vi "CSM - Running Log - DebugTool.vi"(10 "Current Module(\"\" to generate an ID)":string="Debug-LogViewer") -> ()   [LabVIEW 2017]
doc: "CSM overall program running log real-time viewer."
uses:
  Utility/_support/Periodic String Filter Level.ctl
  Utility/Periodic String Filter Setting.ctl
  _Shared/Change Speed Counter.vi
  _Shared/Rising Edge.vi
  _Shared/Debounced Signal.vi
  Communicable State Machine.lvlib
  _Shared/CSM Shared.lvlib
  _Support/csm-tool-support.lvlib
  _csmHelper/API with lvcsm Support/CSM-Helper API with lvcsm Support.lvlib
  addons/Logger/CSM File Logger.lvlib
  _ui/csm-ui-support.lvlib
panel:
  in  "Record.Stop":bool
  in  "Record.Start":bool
  in  "Clear":bool
  in  "BackTop":bool
  in  "Toolbar.History Length(char)":i32=50000 caption="History(char)" min=1000 max=100000000 step=1
  in  "Peroid Logs":bool
  out "State History":string
  in  "Tab":enum32{"Error History", "Broadcast Registry"}(tab)
  out "Error History":string
  out "Broadcast Registry":string[][](table)
  out "LogInQ":i32 caption="LogInQ:"
  out "log handling Speed(#/s)":dbl caption="log handling Speed(#/s):"
  out "LogInQ change(#/s)":dbl caption="LogInQ change(#/s):"
  out "Level":T1 caption="Level:"
  in  "Stop":bool
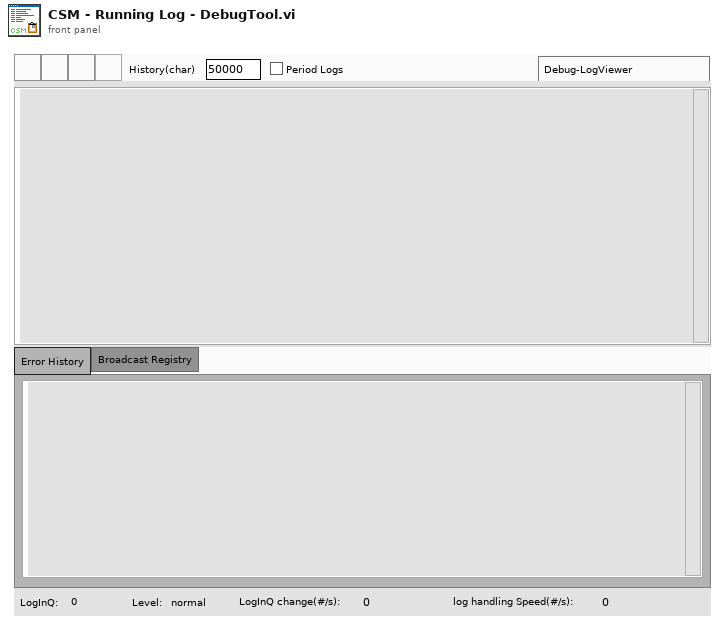
[diagram p1: front panel]
types:
  T1 = typedef "Communicable State Machine.lvlib/Periodic String Filter Level.ctl" = enum16{"normal", "L1", "L2", "L3", "L4"}
  T2 = typedef "Communicable State Machine.lvlib/Periodic String Filter Setting.ctl" = cluster{"threashold(#/s)":dbl, "Check Peroid(s)":dbl}
  T3 = typedef "Communicable State Machine.lvlib/_CSM_GlobalLog_MSG.ctl" = cluster{"Name (\"\" to Use UUID)":string, "Current State":string, "Arguments":string, "Source Message":T4, "Source Module":string, "Complete(T)/Start(F)":bool, "LogType":T5, "Time Stamp":timestamp}
  T4 = typedef "Communicable State Machine.lvlib/_CSM_Response Source Message.ctl" = cluster{"‘State":string, "’Arguments":string, "’Error":errorcluster}
  T5 = typedef "Communicable State Machine.lvlib/_CSM_GlobalLog_MSG_TYPE.ctl" = enum16{"User Log", "State Change", "Status", "Interrupt", "Register", "Unregister", "Error Log", "Module Created", "Module Destroyed", "Async Message", "No-Rep Async Message", "Sync Message"}
  T6 = enum32{"Invalid", "Standard", "Closed", "Hidden", "Minimized", "Maximized"}
  T7 = enum32{"invalid app kind", "Development System", "Run Time System", "Student Edition", "Embedded LabVIEW", "Evaluation", "Custom"}
  T8 = typedef "LVPoint32TypeDef.ctl" = cluster{"Horizontal":i32, "Vertical":i32}
  T9 = cluster{"Shift":bool, "Ctrl":bool, "Alt":bool, "Cmd":bool, "Opt":bool}
  T10 = cluster{"Core":cluster{"Current VI Reference":refnum<vi>, "Close Panel on Exit?":bool}, "Toolbar.Advance":refnum<vi>[], "LoggerWatchDogQueue":refnum<queue>, "LogFile":path}
  T11 = cluster{"Current VI Reference":refnum<vi>, "Close Panel on Exit?":bool}
  T12 = typedef "Communicable State Machine.lvlib/CSM - Broadcast Message Type.ctl" = enum16{"<Null>", "Status", "Interrupt"}
  T13 = cluster{string, "Name":string, "Target CSM":string, "Target State":string, "Register Type":T12}[]
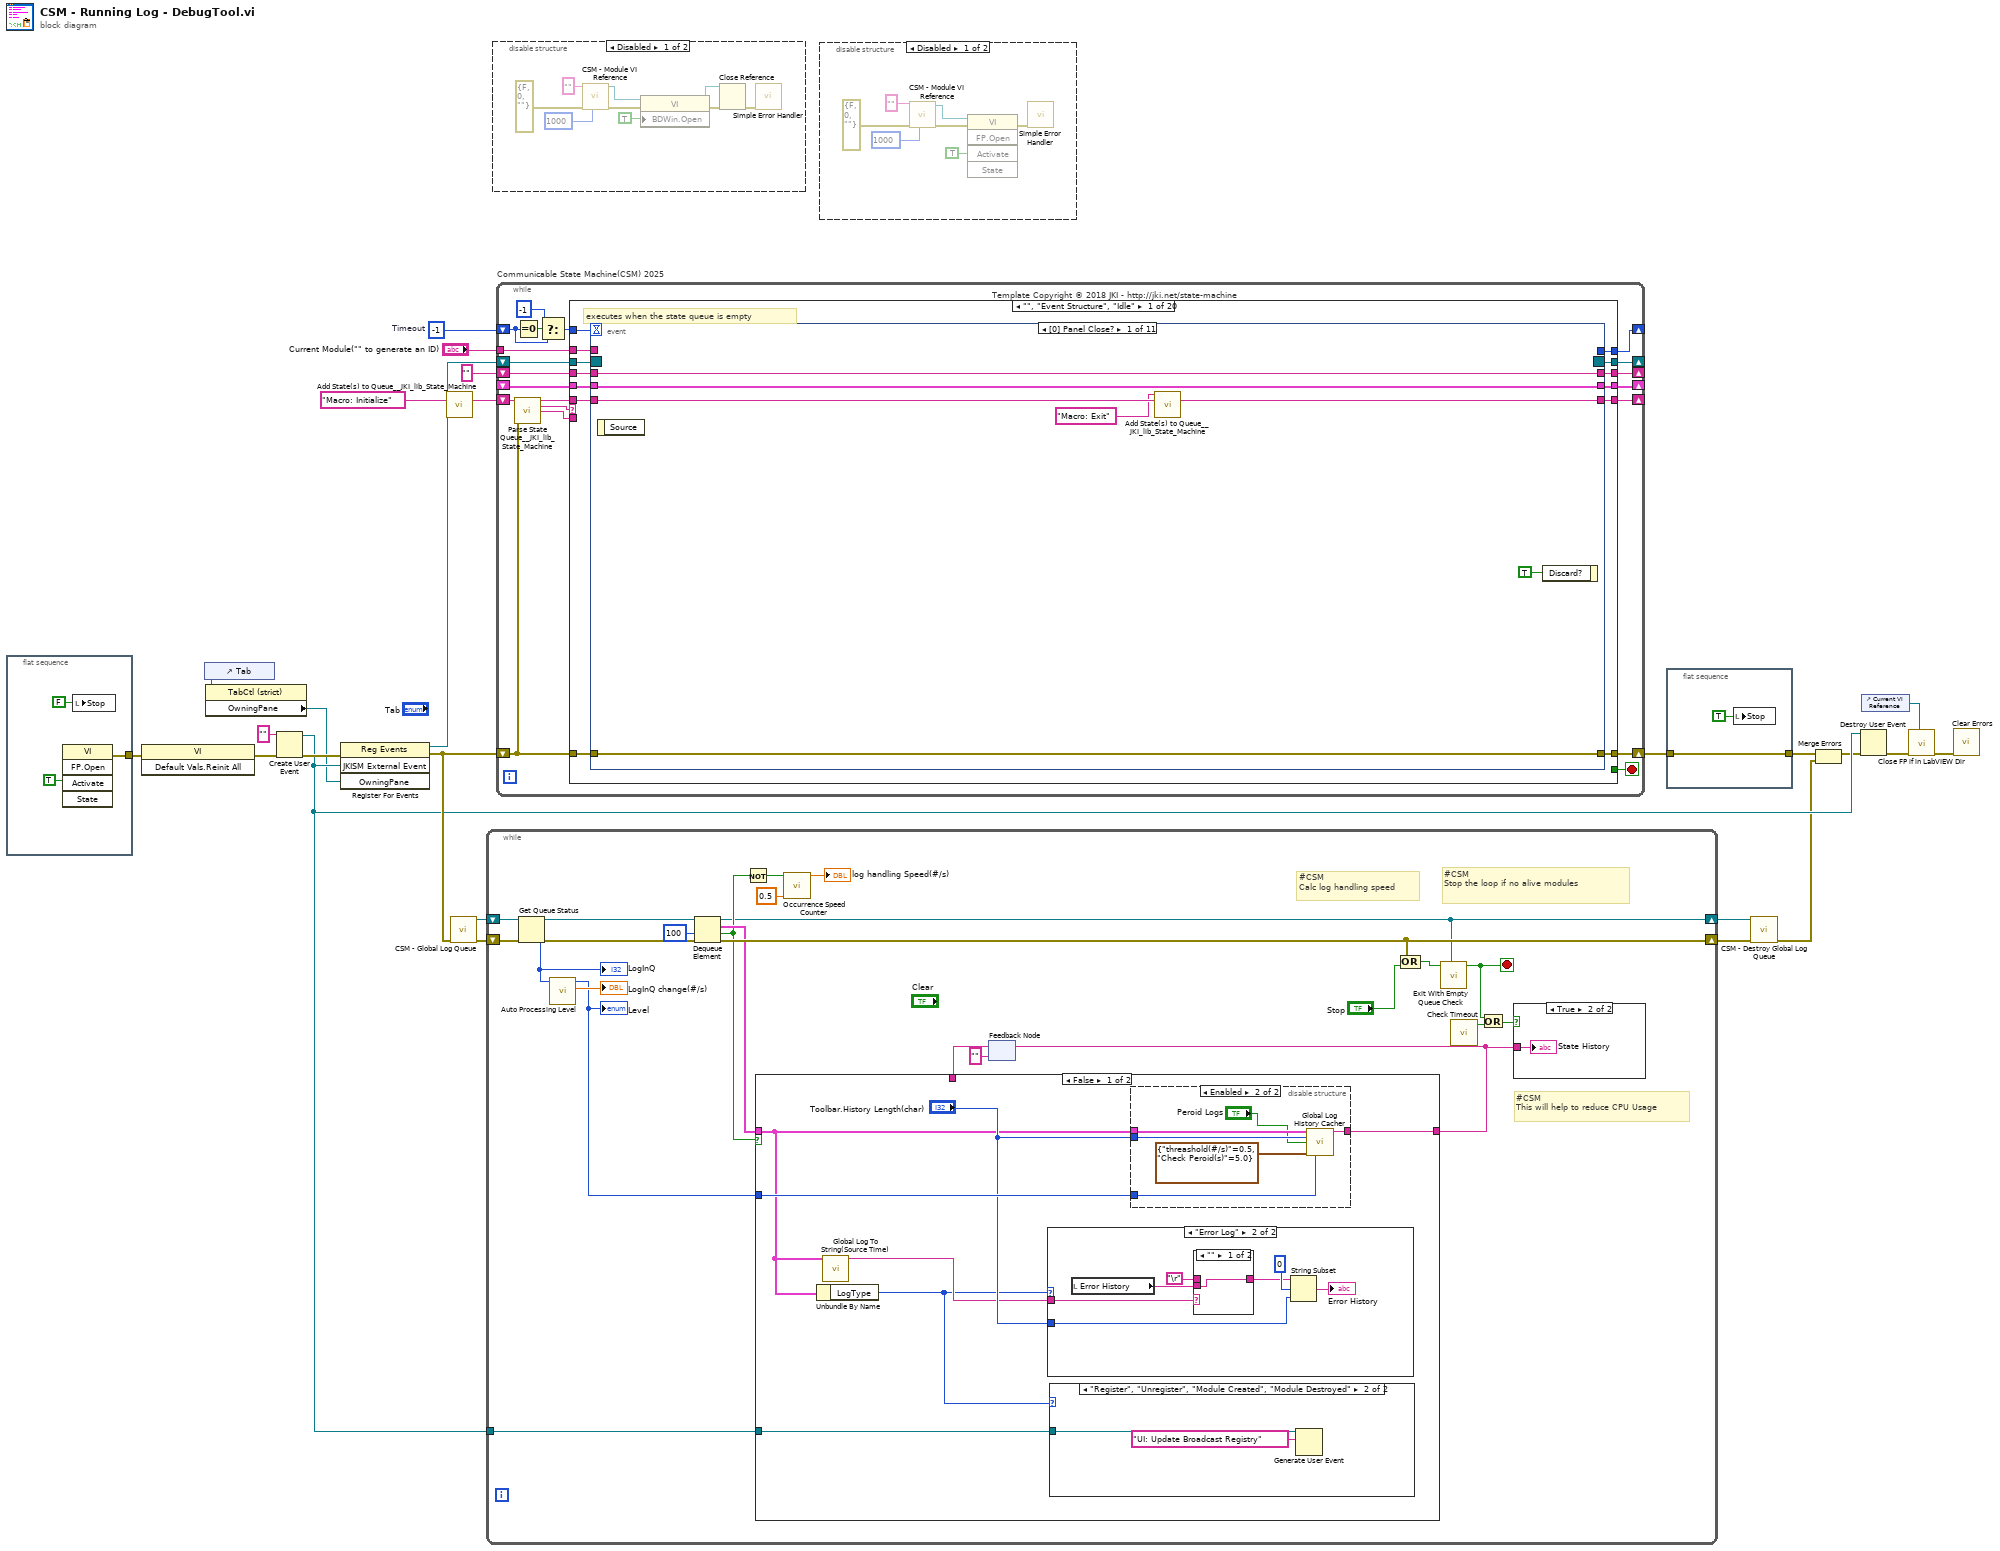
[diagram p0: block diagram]
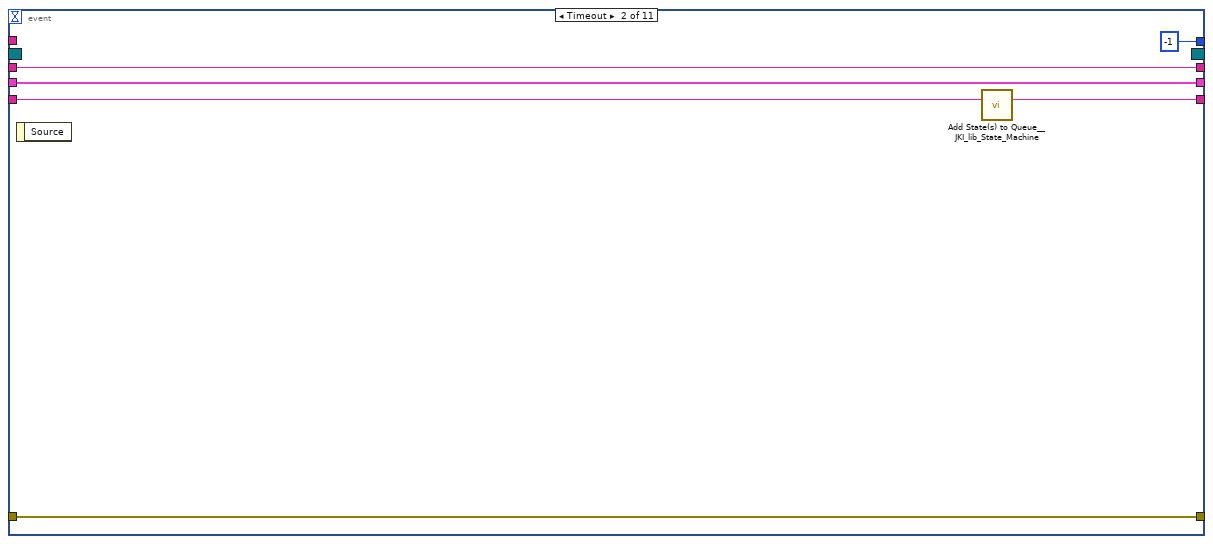
[diagram p4: hidden frame]
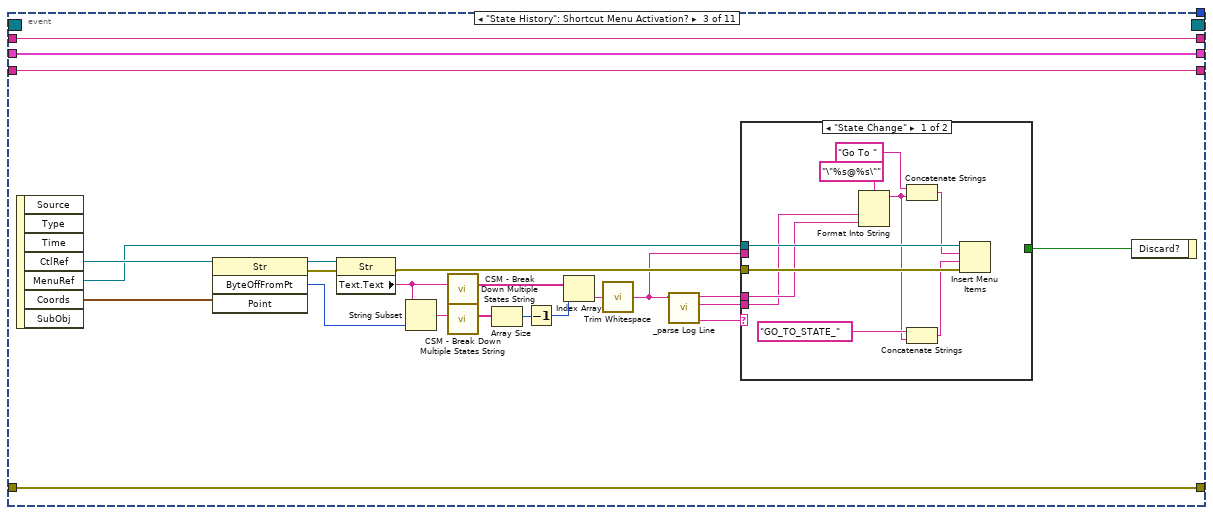
[diagram p5: hidden frame]
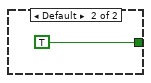
[diagram p6: hidden frame]
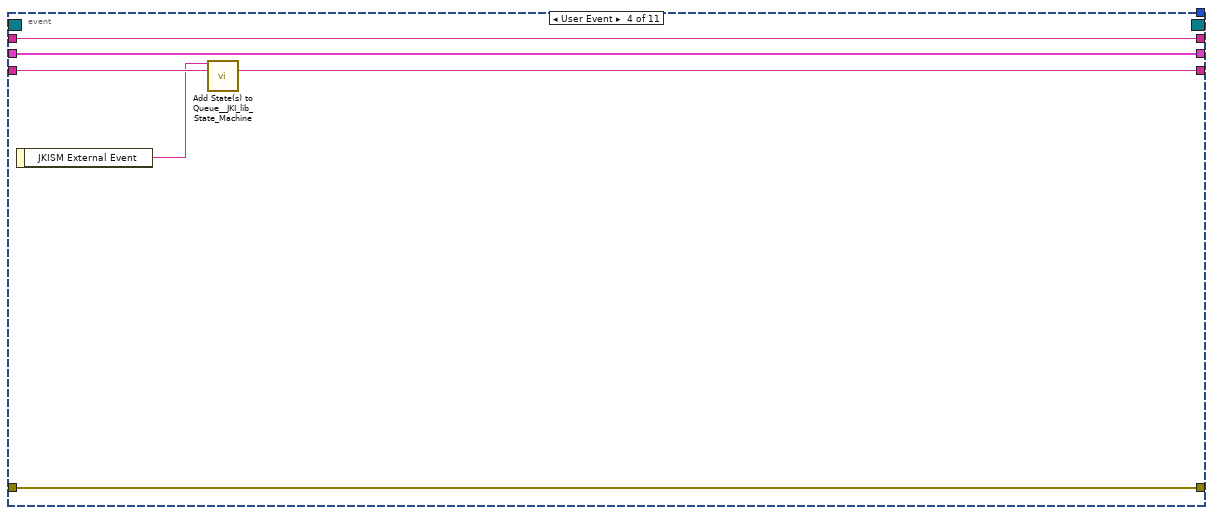
[diagram p7: hidden frame]
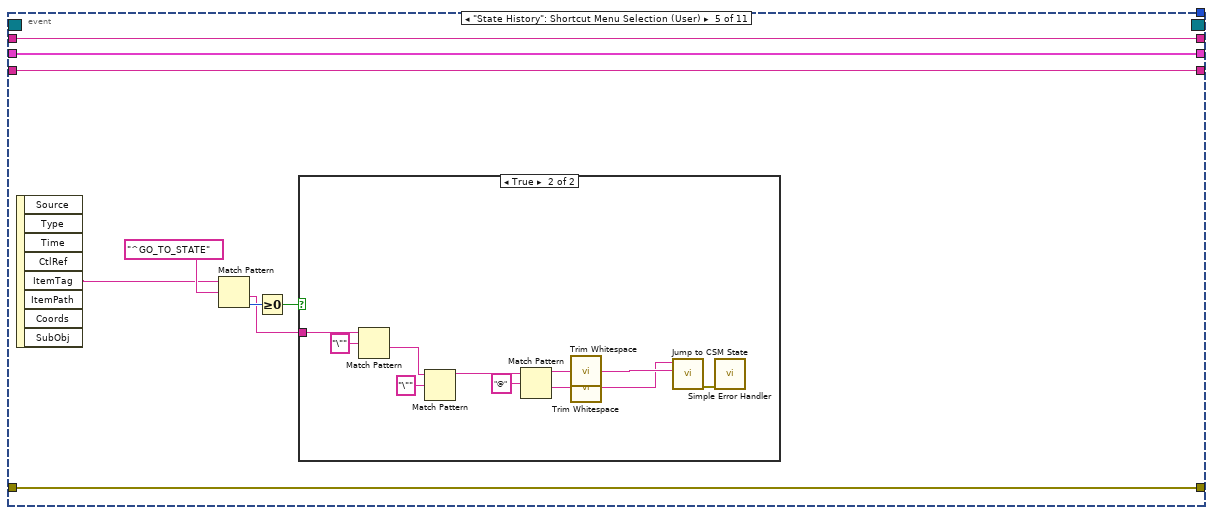
[diagram p8: hidden frame]
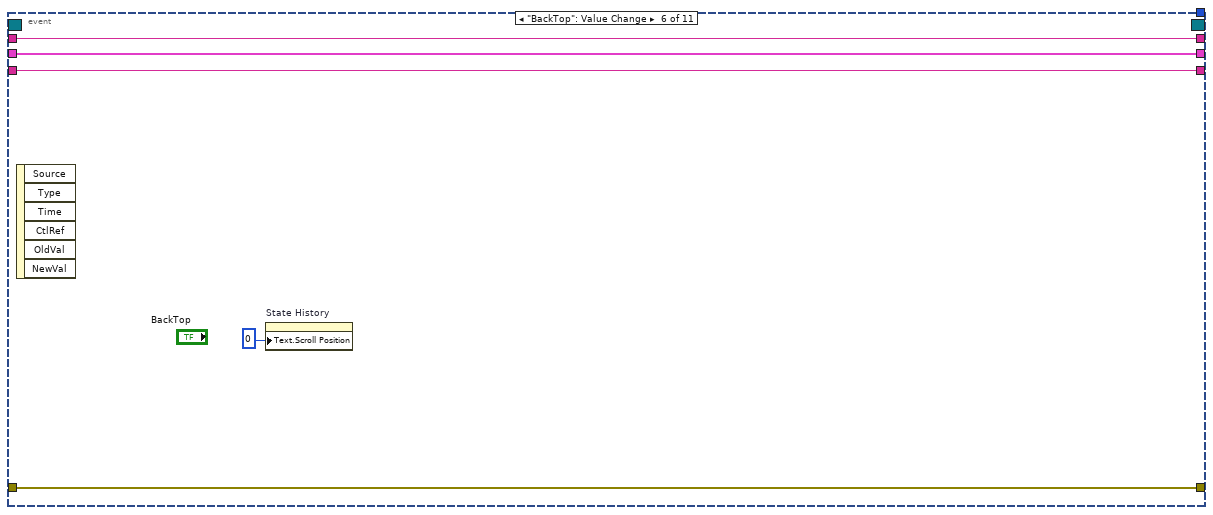
[diagram p10: hidden frame]
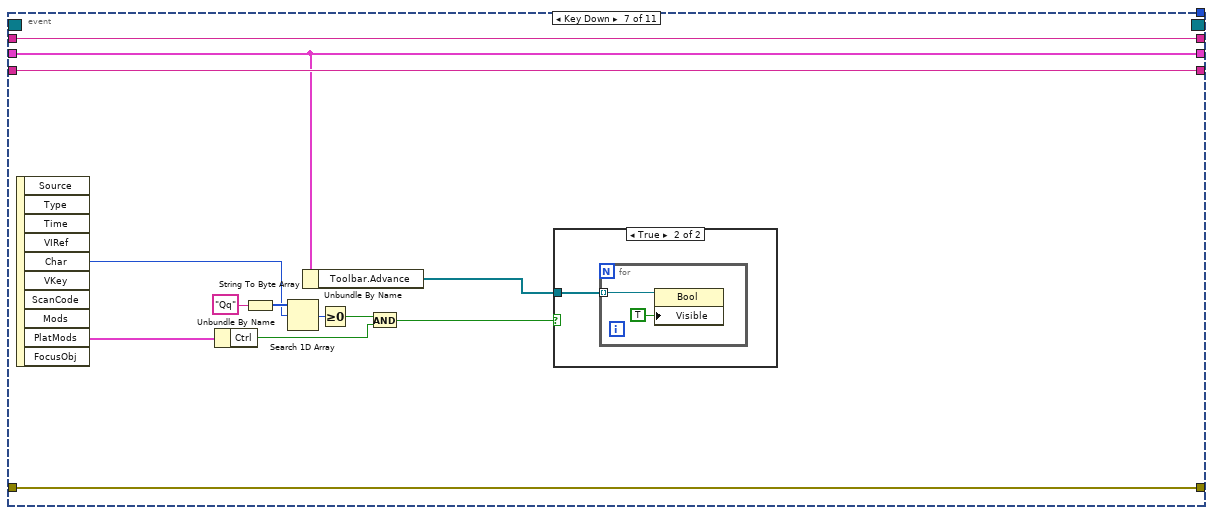
[diagram p11: hidden frame]
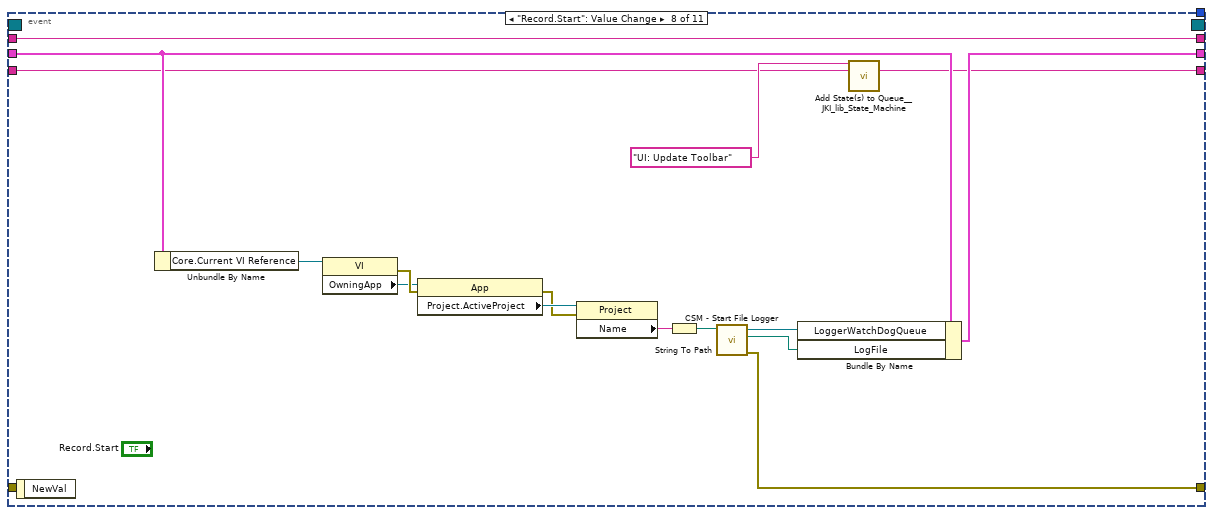
[diagram p13: hidden frame]
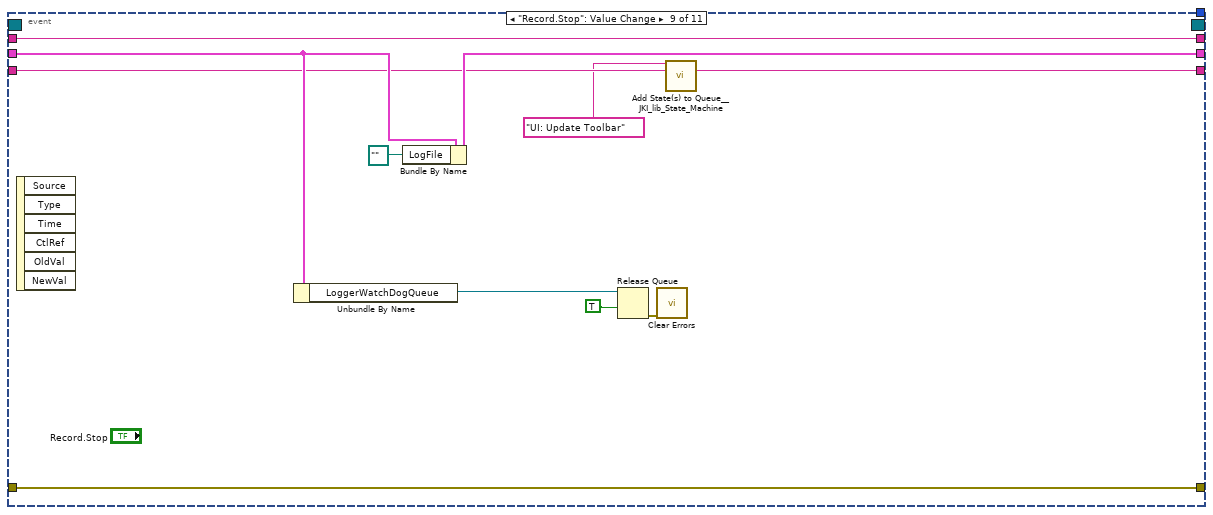
[diagram p14: hidden frame]
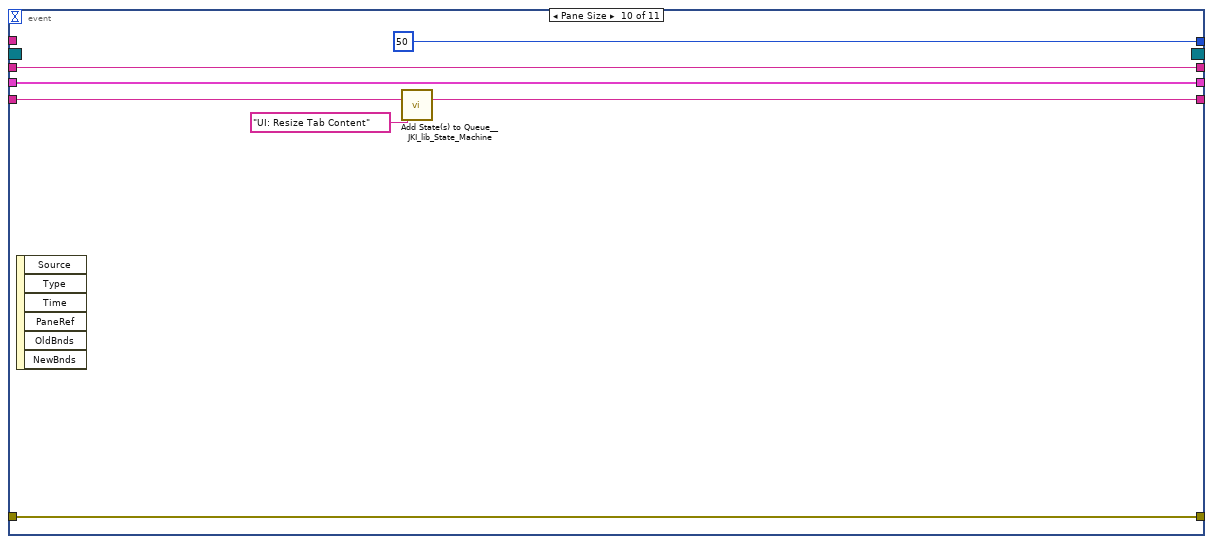
[diagram p15: hidden frame]
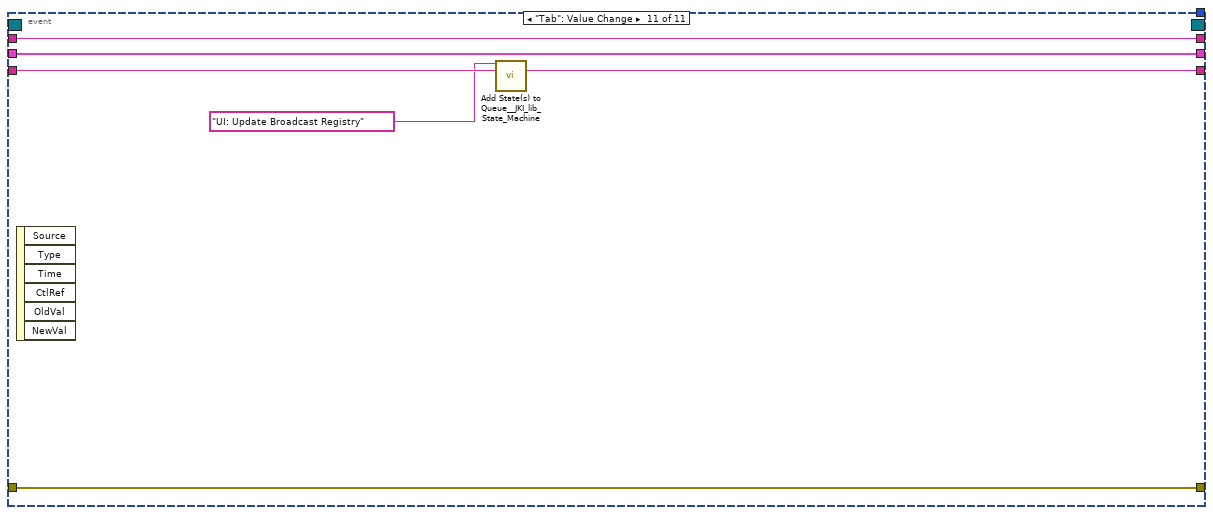
[diagram p16: hidden frame]
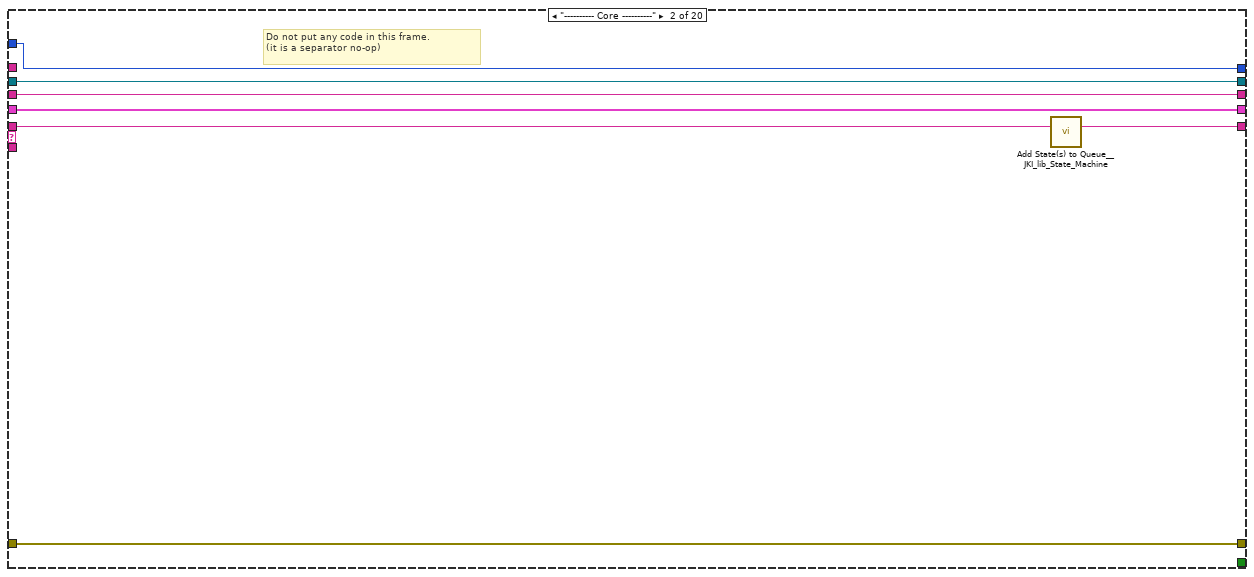
[diagram p17: hidden frame]
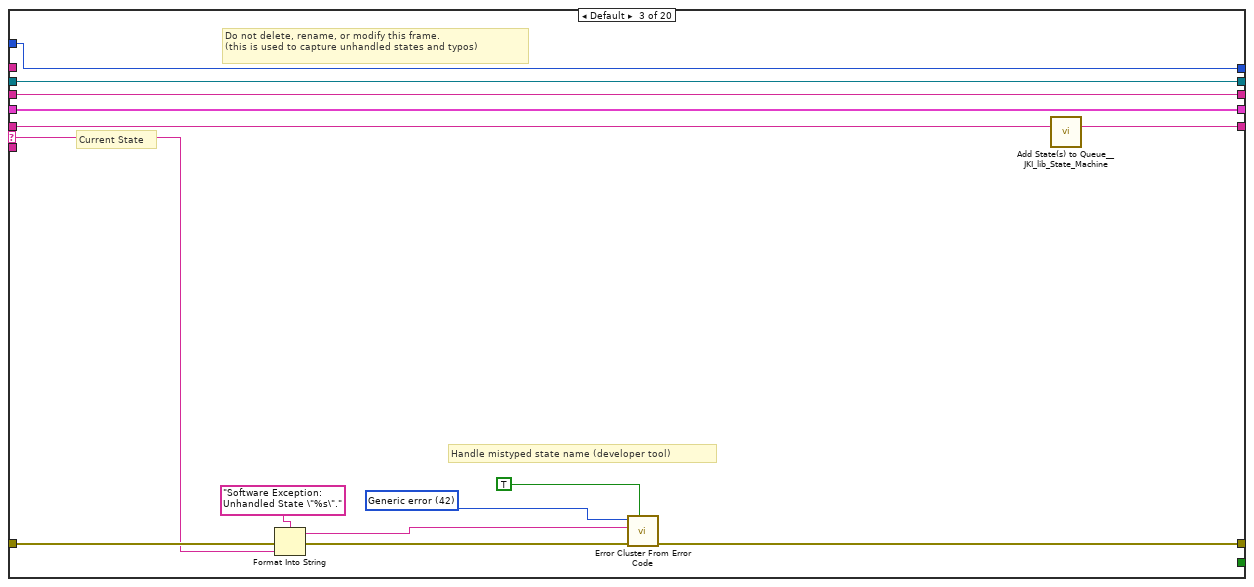
[diagram p18: hidden frame]
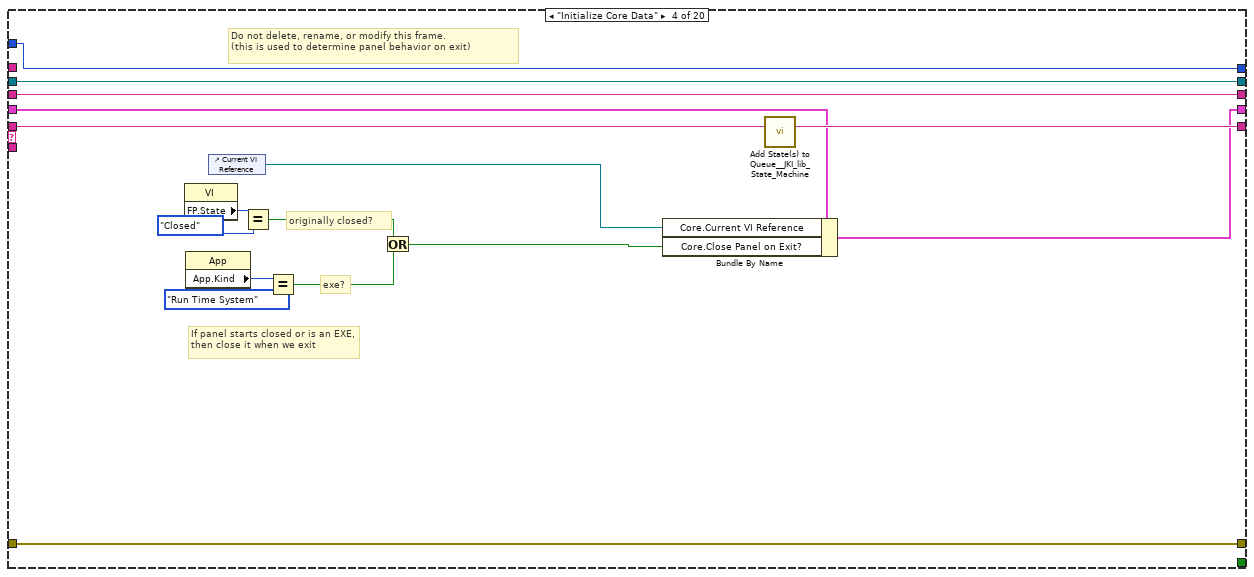
[diagram p19: hidden frame]
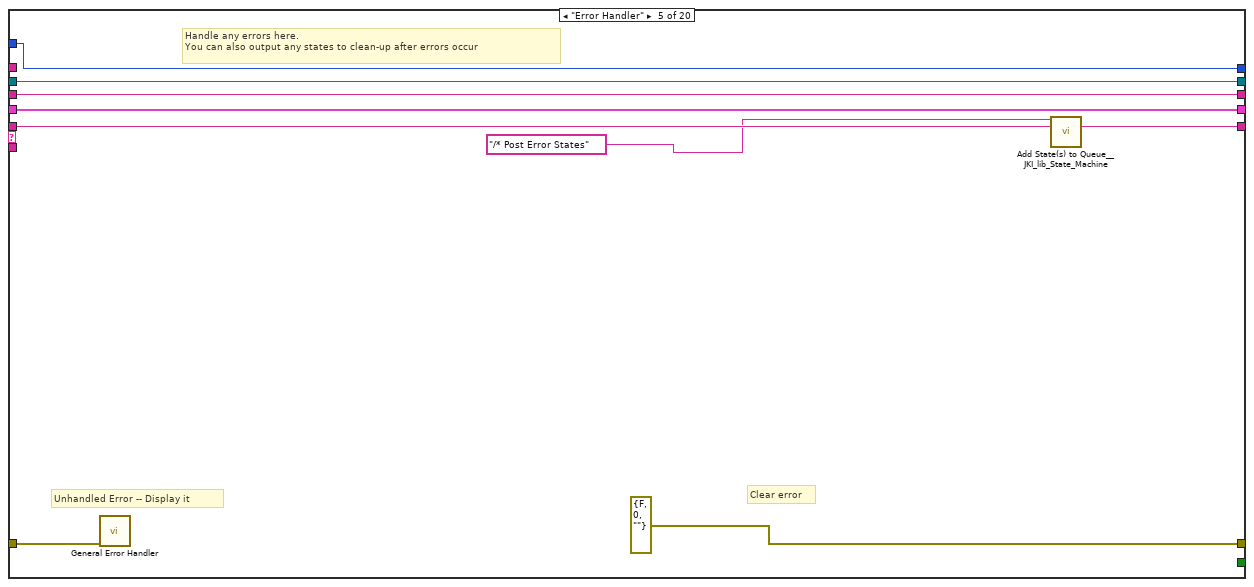
[diagram p20: hidden frame]
diagram:
  w14 = -1  # Timeout
  n1 = flat-sequence {
    tunnel: [w26] -> w6
    frame #0 {
      n2 = invoke class="VI" method="FP.Open"("Activate"=TRUE ("Activate?")) -> (error out=w26:errorcluster)  [unwired: 4 in, 4 out]
      n3 = local write "Stop"(FALSE ("Stop")) -> ()
    }
  }
  n4 = invoke class="VI" method="Default Vals.Reinit All"(error in=w6) -> (error out=w18:errorcluster)  [unwired: 2 in, 2 out]
  n5 = control-ref of="Tab"() -> (w2:refnum<vi>)
  n6 = property class="TabCtl (strict)"(reference=w2) -> ("OwningPane"=w1:refnum<vi>)  [unwired: 1 in, 2 out]
  n7 = Create User Event(user event datatype="" ("JKISM External Event"), error in=w18) -> (user event=w11:refnum<user-event>, error out=w21:errorcluster)
  n8 = register-events(error in=w21, w11, w1) -> (reference out=w17:refnum<event-registration>, error out=w12:errorcluster)  [unwired: 1 in]
  n9 = call <vilib>:"Add State(s) to Queue__JKI_lib_State_Machine.vi"("State(s) in (\"\")"="Macro: Initialize") -> ("States Out"=w20:string)  [unwired: 14 in]
  n10 = call "CSM - Global Log Queue.vi"("Error In"=w12) -> ("error out"=w24:errorcluster, "Global Log Queue"=w22:refnum<queue>)  [unwired: 9 in]
  n11 = while {
    shift-right: [w51] -> w25
    shift-left: w24 -> [w48]
    shift-right: [w38] -> w23
    shift-left: w22 -> [w52]
    tunnel: w11 -> [w30]
    stop <- w31 stop-if-true
    # "#CSM\nCalc log handling speed"
    # "#CSM\nStop the loop if no alive modules"
    # "#CSM\nThis will help to reduce CPU Usage"
    n12 = Get Queue Status(queue=w52, error in (no error)=w48) -> (queue out=w50:refnum<queue>, error out=w49:errorcluster, # elements in queue=w34:i32)  [unwired: 1 in, 5 out]
    "LogInQ" <- w34
    n13 = call "Auto Processing Level.vi"("#Left In Q"=w34) -> ("LogInQ Changing Speed (#/s)"=→"LogInQ change(#/s)":dbl, "Level"=w33:T1)  [unwired: 8 in, 1 out]
    "Level" <- w33
    n14 = Dequeue Element(queue=w50, timeout in ms (-1)=100, error in (no error)=w49) -> (queue out=w38:refnum<queue>, element=w47:T3, timed out?=w40:bool, error out=w51:errorcluster)
    n15 = Not(x=w40) -> (.not. x?=w39:bool)
    n16 = call "Occurrence Speed Counter.vi"("Period (0.1s)"=0.5, "Occured? (T)"=w39) -> ("Speed (#/s)"=→"log handling Speed(#/s)":dbl)  [unwired: 7 in, 2 out]
    n17 = feedback #1("" ("String Cache")) -> (w43:string)
    n18 = case shown="False" w40 {
      tunnel: w47 -> [w56 _]
      tunnel: [w59 w83] -> w44
      tunnel: w43 -> [_ w83]
      tunnel: w33 -> [w58 _]
      tunnel: w30 -> [w53 _]
      frame False {
        n19 = Unbundle By Name(w56) -> ("LogType"=w54:T5)
        n20 = call "Global Log To String(Source Time).vi"("Log"=w56) -> ("Log String"=w55:string)  [unwired: 9 in]
        n21 = case shown="\"Error Log\"" w54 {
          tunnel: w55 -> [_ w63]
          tunnel: "Toolbar.History Length(char)" -> [_ w62]
          frame "User Log", Default {
          }
          frame "Error Log" {
            n22 = local read "Error History"() -> (w67:string)
            n23 = case shown="\"\"" w63 {
              selector: w63 -> [_ w70]
              tunnel: "\r" -> [_ w73]
              tunnel: w67 -> [w69 w72]
              tunnel: [w69 w71] -> w65
              frame "" {
              }
              frame Default {
                n24 = Concatenate Strings(w70, w73, w72) -> (w71:string)
              }
            }
            n25 = String Subset(string=w65, offset (0)=0, length (rest)=w62) -> (substring=→"Error History":string)
          }
        }
        n26 = case shown="\"Register\", \"Unregister\", \"Module Created\", \"Module Destroyed\"" w54 {
          tunnel: w53 -> [_ w61]
          frame "User Log", Default {
          }
          frame "Register", "Unregister", "Module Created", "Module Destroyed" {
            n27 = Generate User Event(user event=w61, event data cluster="UI: Update Broadcast Registry" ("event data")) -> ()  [unwired: 2 in, 2 out]
          }
        }
        n28 = disable-structure shown="Enabled" {
          disable-tunnel: w56 -> [w76 w81]
          disable-tunnel: [w74 w82] -> w59
          disable-tunnel: w58 -> [_ w80]
          disable-tunnel: "Toolbar.History Length(char)" -> [_ w78]
          frame Disabled {
            # "#CSM \nno periodical filter"
            n29 = call "Global Log To String(Source Time).vi"("Log"=w76) -> ("Log String"=w75:string)  [unwired: 9 in]
            n30 = call "String History Cacher.vi"("String"=w75) -> ("String Cache"=w74:string)  [unwired: 10 in]
          }
          frame Enabled {
            n31 = call "Global Log History Cacher.vi"("Global Log Data"=w81, "Length (10000)"=w78, "With Periodic Info? (T)"="Peroid Logs", "Settings"=T2 {"threashold(#/s)"=0.5, "Check Peroid(s)"=5.0}, "Level (Normal)"=w80) -> ("String Cache"=w82:string)  [unwired: 10 in]
          }
        }
      }
      frame True {
      }
    }
    n32 = feedback-in #1(w44) -> ()
    n33 = Compound Arithmetic op=OR(w51, "Stop") -> (w36:bool)
    n34 = call "Exit With Empty Queue Check.vi"("Queue"=w38, "Stop"=w36) -> ("Exit"=w31:bool)  [unwired: 8 in, 1 out]
    n35 = call "Check Timeout.vi"() -> ("Timeout"=w45:bool)  [unwired: 8 in]
    n36 = Or(x=w31, y=w45) -> (x .or. y?=w37:bool)
    n37 = case shown="True" w37 {
      tunnel: w44 -> [_ w84]
      frame False {
      }
      frame True {
        "State History" <- w84
      }
    }
  }
  n38 = disable-structure shown="Disabled" {
    frame Disabled {
      n39 = call "CSM - Module VI Reference.vi"("Response Timeout (-2 Using Global Settings)"=1000 ("Response Timeout(5000 ms)"), "error in (no error)"=errorcluster {"status"=FALSE, "code"=0, "source"=""}, "CSM Name"="") -> ("error out"=w93:errorcluster, "CSM Module VIRef"=w90:refnum<vi>)  [unwired: 7 in]
      n40 = property class="VI"(reference=w90, error in=w93, "BDWin.Open"=TRUE ("Block Diagram Window:Open")) -> (reference out=w91:refnum<vi>, error out=w92:errorcluster)
      n41 = Close Reference(reference=w91, error in (no error)=w92) -> (error out=w89:errorcluster)
      n42 = call <vilib>:"Simple Error Handler.vi"("error in (no error)"=w89) -> ()  [unwired: 4 in, 5 out]
    }
    frame Enabled {
    }
  }
  n43 = while "Communicable State Machine(CSM) 2025" {
    shift-right: [w106] -> _
    shift-left: _ -> [w105]
    shift-right: [w109] -> w7
    shift-left: w12 -> [w104]
    shift-right: [w108] -> _
    shift-left: w20 -> [w110]
    shift-right: [w102] -> _
    shift-left: w17 -> [w103]
    tunnel: "Current Module(\"\" to generate an ID)" -> [w101]
    shift-right: [w99] -> _
    shift-left: "" ("String Cache") -> [w100]
    shift-right: [w98] -> _
    shift-left: w14 -> [w95]
    stop <- w107 stop-if-true
    # "Template Copyright © 2018 JKI - http://jki.net/state-machine"
    n44 = call <vilib>:"Parse State Queue__JKI_lib_State_Machine.vi"("State Queue"=w110, "Error In (no error)"=w104) -> ("Remaining States"=w112:string, "Current State"=w113:string, "Arguments"=w111:string)  [unwired: 11 in]
    n45 = Equal To 0?(x=w95) -> (x = 0?=w97:bool)
    n46 = Select(t=-1 ("Timeout"), s=w97, f=w95) -> (s? t:f=w96:i32)
    n47 = case shown="\"\", \"Event Structure\", \"Idle\"" w113 {
      selector: w113 -> [_ _ w271 _ _ _ _ _ _ _ _ _ _ _ _ _ _ _ _ _]
      tunnel: w112 -> [w126 w267 w275 w297 w306 w314 w321 w332 w338 w347 w354 w363 w375 w389 w461 w490 w507 w517 w525 w534]
      tunnel: w111 -> [_ _ _ _ _ _ _ _ _ _ _ _ w370 w383 _ _ _ _ _ _]
      tunnel: w105 -> [w124 w264 w273 w290 w303 w312 w318 _ w337 w342 w351 w358 w373 w385 w460 w485 w506 w514 w522 w531]
      tunnel: [w123 w265 w277 w294 errorcluster {"status"=FALSE, "code"=0, "source"=""} ("error out") w311 w319 w329 w334 w343 w352 w361 w371 w386 w462 w491 w508 w515 w523 w532] -> w109
      tunnel: w104 -> [w122 w265 w276 w294 w302 w311 w319 w329 w334 w344 w352 w361 w372 w387 w462 w491 w508 w515 w523 w532]
      tunnel: [w125 w266 w274 w296 w305 w313 w320 w331 w338 w346 w353 w362 w374 w388 w461 w490 w507 w516 w524 w533] -> w108
      tunnel: [_ _ _ _ _ TRUE _ _ _ _ _ _ _ _ _ _ _ _ _ _] -> w107
      tunnel: [w121 w264 w273 w295 w303 w312 w318 w330 w337 w342 w351 w358 w373 w385 w460 w485 w506 w514 w522 w531] -> w106
      tunnel: w96 -> [w120 w261 w268 w282 w298 w307 w315 w322 w333 w339 w348 w355 w367 w380 w455 w471 w503 w511 w518 w526]
      tunnel: w103 -> [w119 w263 w270 w284 w300 w309 w317 w327 w336 w341 w350 w360 w369 w382 w459 w489 w505 w513 w520 w528]
      tunnel: [w118 w263 w270 w284 w300 w309 w317 w327 w336 w341 w350 w360 w369 w382 w459 w489 w505 w513 w520 w528] -> w102
      tunnel: w101 -> [w117 _ _ _ _ _ _ _ _ _ _ _ _ _ _ _ _ _ _ _]
      tunnel: w100 -> [w116 w262 w269 w283 w299 w308 w316 w326 w335 w340 w349 w359 w368 w381 w458 w488 w504 w512 w519 w527]
      tunnel: [w115 w262 w269 w283 w299 w308 w316 w326 w335 w340 w349 w359 w368 w381 w458 w488 w504 w512 w519 w527] -> w99
      tunnel: [w114 w261 w268 w282 w298 w307 w315 w322 w333 w339 w348 w355 w367 w380 w455 w471 w503 w511 w518 w526] -> w98
      frame "", "Event Structure", "Idle" {
        # "executes when the state queue is empty"
        n48 = event shown="[0] Panel Close?" {
          selector: w119 -> [_ _ _ _ _ _ _ _ _ _ _]
          dyn-events: [_ _ _ _ _ _ _ _ _ _ _] -> w118
          timeout: w120 -> [_ _ _ _ _ _ _ _ _ _ _]
          tunnel: w126 -> [w133 w139 w162 w175 w188 w204 w217 w222 w239 w250 w256]
          tunnel: [w132 w138 w162 w176 w188 w204 w217 w221 w238 w251 w257] -> w125
          tunnel: w124 -> [w130 w136 w160 w178 w186 w202 w207 w231 w245 w253 w259]
          tunnel: [w131 w137 w161 w179 w187 w203 w216 w233 w247 w254 w260] -> w123
          tunnel: w122 -> [w131 w137 w161 w179 w187 w203 w216 _ w247 w254 w260]
          tunnel: [w130 w136 w160 w178 w186 w202 w207 w234 w241 w253 w259] -> w121
          tunnel: w117 -> [_ _ _ _ _ _ _ _ _ _ _]
          tunnel: w116 -> [w127 w135 w159 w177 w185 w201 w215 w236 w246 w252 w258]
          tunnel: [w127 w135 w159 w177 w185 w201 w215 w236 w246 w252 w258] -> w115
          tunnel: [_ -1 ("Timeout") _ _ _ _ _ _ _ 50 ("Timeout") _] -> w114
          event Panel Close? {
            n49 = event-data() -> ()  [unwired: 1 in, 1 out]
            n50 = call <vilib>:"Add State(s) to Queue__JKI_lib_State_Machine.vi"("State(s) in Front (\"\")"="Macro: Exit", "State(s) in (\"\")"=w133) -> ("States Out"=w132:string)  [unwired: 13 in]
            n51 = event-data("Discard?"=TRUE) -> ()  [unwired: 1 in, 1 out]
          }
          event Timeout {
            n52 = event-data() -> ()  [unwired: 1 in, 1 out]
            n53 = call <vilib>:"Add State(s) to Queue__JKI_lib_State_Machine.vi"("State(s) in (\"\")"=w139) -> ("States Out"=w138:string)  [unwired: 14 in]
          }
          event "State History": Shortcut Menu Activation? {
            n54 = event-data() -> ("CtlRef"=w142:refnum<vi>, "MenuRef"=w141:refnum<k9>, "Coords"=w140:T8)  [unwired: 1 in, 4 out]
            n55 = invoke class="Str" method="ByteOffFromPt"(reference=w142, "Point"=w140) -> (reference out=w158:refnum<vi>, error out=w156:errorcluster, "ByteOffFromPt"=w157:i32)  [unwired: 2 in, 1 out]
            n56 = property class="Str"(reference=w158, error in=w156) -> (error out=w148:errorcluster, "Text.Text"=w154:string)  [unwired: 1 out]
            n57 = String Subset(string=w154, length (rest)=w157) -> (substring=w155:string)  [unwired: 1 in]
            n58 = call "CSM - Break Down Multiple States String.vi"("States"=w154) -> ("Multiple States"=w153:string[])  [unwired: 10 in]
            n59 = call "CSM - Break Down Multiple States String.vi"("States"=w155) -> ("Multiple States"=w152:string[])  [unwired: 10 in]
            n60 = Array Size(array=w152) -> (size(s)=w151:i32)
            n61 = Decrement(x=w151) -> (x-1=w150:i32)
            n62 = Index Array(array=w153, index=w150) -> (element=w149:string)
            n63 = call <vilib>:"Trim Whitespace.vi"("string"=w149) -> ("trimmed string"=w147:string)  [unwired: 1 in]
            n64 = call "_parse Log Line.vi"("String"=w147) -> ("LogType"=w146:string, "State"=w144:string, "CSM"=w145:string)  [unwired: 8 in]
            n65 = case shown="\"State Change\"" w146 {
              tunnel: w141 -> [w172 _]
              tunnel: w147 -> [_ _]
              tunnel: w148 -> [w170 _]
              tunnel: [_ TRUE] -> w143
              tunnel: w145 -> [w168 _]
              tunnel: w144 -> [w167 _]
              frame "State Change" {
                n66 = Format Into String(format string="\"%s@%s\"", w167, w168) -> (resulting string=w163:string)  [unwired: 2 in, 1 out]
                n67 = Concatenate Strings("Go To " ("format string"), w163) -> (w166:string)
                n68 = Concatenate Strings("GO_TO_STATE_" ("item tags"), w163) -> (w164:string)
                n69 = Insert Menu Items(6:w170, 7:w164, 8:w166, 9:w172) -> ()  [unwired: 2 in, 3 out]
              }
              frame Default {
              }
            }
            n70 = event-data("Discard?"=w143) -> ()  [unwired: 1 in, 1 out]
          }
          event User Event {
            n71 = event-data() -> ("JKISM External Event"=w174:string)  [unwired: 1 in]
            n72 = call <vilib>:"Add State(s) to Queue__JKI_lib_State_Machine.vi"("State(s) in Front (\"\")"=w174, "State(s) in (\"\")"=w175) -> ("States Out"=w176:string)  [unwired: 13 in]
          }
          event "State History": Shortcut Menu Selection (User) {
            n73 = event-data() -> ("ItemTag"=w180:string)  [unwired: 1 in, 7 out]
            n74 = Match Pattern(string=w180, regular expression="^GO_TO_STATE") -> (after substring=w181:string, offset past match=w183:i32)  [unwired: 1 in, 2 out]
            n75 = Greater Or Equal To 0?(x=w183) -> (x >= 0?=w182:bool)
            n76 = case shown="True" w182 {
              tunnel: w181 -> [_ w199]
              frame False {
              }
              frame True {
                n77 = Match Pattern(string=w199, regular expression="\"") -> (after substring=w196:string)  [unwired: 1 in, 3 out]
                n78 = Match Pattern(string=w196, regular expression="\"") -> (before substring=w195:string)  [unwired: 1 in, 3 out]
                n79 = Match Pattern(string=w195, regular expression="@") -> (before substring=w193:string, after substring=w192:string)  [unwired: 1 in, 2 out]
                n80 = call <vilib>:"Trim Whitespace.vi"("string"=w193) -> ("trimmed string"=w191:string)  [unwired: 1 in]
                n81 = call <vilib>:"Trim Whitespace.vi"("string"=w192) -> ("trimmed string"=w190:string)  [unwired: 1 in]
                n82 = call "Jump to CSM State.vi"("State"=w191, "Name"=w190) -> ("error out"=w189:errorcluster)  [unwired: 9 in]
                n83 = call <vilib>:"Simple Error Handler.vi"("error in (no error)"=w189) -> ()  [unwired: 4 in, 5 out]
              }
            }
          }
          event "BackTop": Value Change {
            n84 = event-data() -> ()  [unwired: 1 in, 6 out]
            n85 = property on="State History" class="Str"("Text.Scroll Position"=u32 0) -> ()  [unwired: 2 in, 2 out]
          }
          event Key Down {
            n86 = event-data() -> ("Char"=w205:i16, "PlatMods"=w210:T9)  [unwired: 1 in, 8 out]
            n87 = Unbundle By Name(w210) -> ("Ctrl"=w209:bool)
            n88 = String To Byte Array(string="Qq") -> (unsigned byte array=w212:u8[])
            n89 = Search 1D Array(1D array=w212, element=w205) -> (index of element=w213:i32)  [unwired: 1 in]
            n90 = Unbundle By Name(w207) -> ("Toolbar.Advance"=w206:refnum<vi>[])
            n91 = Greater Or Equal To 0?(x=w213) -> (x >= 0?=w214:bool)
            n92 = And(x=w214, y=w209) -> (x .and. y?=w208:bool)
            n93 = case shown="True" w208 {
              tunnel: w206 -> [_ w218]
              frame False {
              }
              frame True {
                n94 = for {
                  tunnel: w218 -> [w220] mode=indexing
                  n95 = property class="Bool"(reference=w220, "Visible"=TRUE) -> ()  [unwired: 1 in, 2 out]
                }
              }
            }
          }
          event "Record.Start": Value Change {
            n96 = event-data() -> ()  [unwired: 1 in, 1 out]
            n97 = Unbundle By Name(w231) -> ("Core.Current VI Reference"=w230:refnum<vi>)
            n98 = property class="VI"(reference=w230) -> (error out=w229:errorcluster, "OwningApp"=w228:refnum<vi>)  [unwired: 1 in, 1 out]
            n99 = property class="App"(reference=w228, error in=w229) -> (error out=w226:errorcluster, "Project.ActiveProject"=w227:refnum<vi>)  [unwired: 1 out]
            n100 = property class="Project"(reference=w227, error in=w226) -> ("Name"=w225:string)  [unwired: 2 out]
            n101 = String To Path(string=w225) -> (path=w224:path)
            n102 = call "CSM - Start File Logger.vi"("Log File Path"=w224) -> ("error out"=w233:errorcluster, "Log File"=w232:path, "Watchdog Queue"=w235:refnum<queue>)  [unwired: 8 in]
            n103 = Bundle By Name(cluster=w231, "LoggerWatchDogQueue"=w235, "LogFile"=w232) -> (w234:T10)
            n104 = call <vilib>:"Add State(s) to Queue__JKI_lib_State_Machine.vi"("State(s) in Front (\"\")"="UI: Update Toolbar" ("State(s) in Front (\"\")"), "State(s) in (\"\")"=w222) -> ("States Out"=w221:string)  [unwired: 13 in]
          }
          event "Record.Stop": Value Change {
            n105 = event-data() -> ()  [unwired: 1 in, 6 out]
            n106 = Unbundle By Name(w245) -> ("LoggerWatchDogQueue"=w244:refnum<queue>)
            n107 = Bundle By Name(cluster=w245, "LogFile"=path "") -> (w241:T10)
            n108 = Release Queue(queue=w244, force destroy? (F)=TRUE) -> (error out=w242:errorcluster)  [unwired: 1 in, 2 out]
            n109 = call <vilib>:"Clear Errors.vi"("error in (no error)"=w242) -> ()  [unwired: 5 in, 2 out]
            n110 = call <vilib>:"Add State(s) to Queue__JKI_lib_State_Machine.vi"("State(s) in Front (\"\")"="UI: Update Toolbar" ("State(s) in Front (\"\")"), "State(s) in (\"\")"=w239) -> ("States Out"=w238:string)  [unwired: 13 in]
          }
          event Pane Size {
            n111 = event-data() -> ()  [unwired: 1 in, 6 out]
            n112 = call <vilib>:"Add State(s) to Queue__JKI_lib_State_Machine.vi"("State(s) in (\"\")"=w250, "State(s) at Back (\"\")"="UI: Resize Tab Content" ("State(s) in Front (\"\")")) -> ("States Out"=w251:string)  [unwired: 13 in]
          }
          event "Tab": Value Change {
            n113 = event-data() -> ()  [unwired: 1 in, 6 out]
            n114 = call <vilib>:"Add State(s) to Queue__JKI_lib_State_Machine.vi"("State(s) in Front (\"\")"="UI: Update Broadcast Registry" ("State(s) in Front (\"\")"), "State(s) in (\"\")"=w256) -> ("States Out"=w257:string)  [unwired: 13 in]
          }
        }
      }
      frame "---------- Core ----------" {
        # "Do not put any code in this frame.\n(it is a separator no-op)"
        n115 = call <vilib>:"Add State(s) to Queue__JKI_lib_State_Machine.vi"("State(s) in (\"\")"=w267) -> ("States Out"=w266:string)  [unwired: 14 in]
      }
      frame Default {
        w280 = 42 items=["No error", "Argument error", "Memory is full", "Out of zone", "End of file", "File already open", "Generic file I/O error", "File not found", "File permission error", "Disk is full", "Duplicate path", "Too many files open", "System feature not enabled", "Resource file not found", "Cannot add resource", "Resource not found", "Image not found", "Image memory error", "Pen does not exist", "Config type invalid", "Config token not found", "Config parse error", "Config memory error", "Bad external code format", "Bad external code offset", "External code not present", "Null window", "Destroy window error", "Null menu", "Print aborted", "Bad print record", "Print driver error", "Windows error during printing", "Memory error during printing", "Print dialog error", "Generic print error", "Invalid device refnum", "Device not found", "Device parameter error", "Device unit error", "Cannot open device", "Device call aborted", "Generic error", "Cancelled by user", "Object ID too low", "Object ID too high", "Object not in heap", "Unknown heap", "Unknown object (invalid DefProc)", "Unknown object (DefProc not in table)", "Message out of range", "Invalid (null) method", "Unknown message", "Manager call not supported", "Bad address", "Network operation in progress", "Network operation timed out", "Connection is busy", "Network attribute not supported", "Network error", "Address in use", "System out of memory", "Connection aborted", "Connection refused", "Not connected", "Already connected", "Connection closed", "Initialization error (interapplication manager)", "Bad occurrence", "Wait on unbound occurrence handler", "Occurrence queue overflow", "Datalog type conflict", "Unused", "Unrecognized type (interapplication manager)", "Memory corrupt", "Failed to make temporary DLL", "Old CIN version", "Drag socket not found", "Failed to load drop-object", "Failed to register OLE object", "Failed to release OLE object", "Format specifier type mismatch", "Unknown format specifier", "Too few format specifiers", "Too many format specifiers", "Scan failed", "Newer CIN version", "Error converting to variant", "Runtime menu error", "Password tampered", "Variant attribute not found", "Incompatible variant data type", "Event data is not available", "Event Store is not present", "Occurrence is not found", "Event Queue is not created", "Event info is not available", "Refnum passed is NULL", "Error retrieving Class GUID", "Error retrieving CoClass GUID", "Error retrieving TypeLib GUID.", "Bad built application magic bytes.", "Specific driver is different from the specific driver associated with the Logical Name.", "There is no session opened to the class driver.", "Max Error", "MAX - Error with config objects", "MAX - Error loading configuration", "MAX - Group not supported"]
        # "Current State"
        # "Do not delete, rename, or modify this frame.\n(this is used to capture unhandled states and typos)"
        # "Handle mistyped state name (developer tool)"
        n116 = Format Into String(format string="Software Exception: Unhandled State \"%s\"." ("message"), error in=w276, w271) -> (resulting string=w279:string, error out=w278:errorcluster)  [unwired: 1 in]
        n117 = call <vilib>:"Error Cluster From Error Code.vi"("show call chain? (False)"=TRUE, "error in (no error)"=w278, "error message (\"\")"=w279, "error code (0)"=w280) -> ("error out"=w277:errorcluster)  [unwired: 5 in]
        n118 = call <vilib>:"Add State(s) to Queue__JKI_lib_State_Machine.vi"("State(s) in (\"\")"=w275) -> ("States Out"=w274:string)  [unwired: 14 in]
      }
      frame "Initialize Core Data" {
        # "Do not delete, rename, or modify this frame.\n(this is used to determine panel behavior on exit)"
        # "originally closed?"
        # "exe?"
        # "If panel starts closed or is an EXE, then close it when we exit"
        n119 = property class="VI"() -> ("FP.State"=w287:T6)  [unwired: 2 in, 2 out]
        n120 = property class="App"() -> ("App.Kind"=w293:T7)  [unwired: 2 in, 2 out]
        n121 = control-ref of="Current VI Reference"() -> (w288:refnum<vi>)
        n122 = Equal?(x=w287, y=T6."Closed" ("Front Panel Window:State")) -> (x = y?=w285:bool)
        n123 = Equal?(x=w293, y=T7."Run Time System" ("Application:Kind")) -> (x = y?=w291:bool)
        n124 = Or(x=w285, y=w291) -> (x .or. y?=w289:bool)
        n125 = Bundle By Name(cluster=w290, "Core.Current VI Reference"=w288, "Core.Close Panel on Exit?"=w289) -> (w295:T10)
        n126 = call <vilib>:"Add State(s) to Queue__JKI_lib_State_Machine.vi"("State(s) in (\"\")"=w297) -> ("States Out"=w296:string)  [unwired: 14 in]
      }
      frame "Error Handler" {
        # "Unhandled Error -- Display it"
        # "Handle any errors here.\nYou can also output any states to clean-up after errors occur"
        # "Clear error"
        n127 = call <vilib>:"General Error Handler.vi"("error in (no error)"=w302) -> ()  [unwired: 10 in, 5 out]
        n128 = call <vilib>:"Add State(s) to Queue__JKI_lib_State_Machine.vi"("State(s) in Front (\"\")"="/* Post Error States", "State(s) in (\"\")"=w306) -> ("States Out"=w305:string)  [unwired: 13 in]
      }
      frame "Exit" {
        # "Do not put any code in this frame.\n(No errors that occur here will be handled.)"
        n129 = call <vilib>:"Add State(s) to Queue__JKI_lib_State_Machine.vi"("State(s) in (\"\")"=w314) -> ("States Out"=w313:string)  [unwired: 14 in]
      }
      frame "---------- Data ----------" {
        # "Do not put any code in this frame.\n(It is a separator no-op. You can make a copy of this frame to create a new Data frame)"
        n130 = call <vilib>:"Add State(s) to Queue__JKI_lib_State_Machine.vi"("State(s) in (\"\")"=w321) -> ("States Out"=w320:string)  [unwired: 14 in]
      }
      frame "Data: Initialize" {
        w323 = refnum<queue> refnum  # LoggerWatchDogQueue
        w324 = path ""  # LogFile
        w325 = refnum<vi>[] []  # Toolbar.Advance
        w328 = T11 {"Current VI Reference"=refnum, "Close Panel on Exit?"=FALSE}  # Core
        # "Data names and types of shift register data are defined by this bundle."
        # "Initialize the shift-register data, here.\n(data names are defined by what you wire into the bundle function)"
        n131 = Bundle("Core"=w328, "Toolbar.Advance"=w325, "LoggerWatchDogQueue"=w323, "LogFile"=w324) -> (w330:T10)  [unwired: 1 in]
        n132 = call <vilib>:"Add State(s) to Queue__JKI_lib_State_Machine.vi"("State(s) in (\"\")"=w332) -> ("States Out"=w331:string)  [unwired: 14 in]
      }
      frame "Data: Initialize References" {
      }
      frame "Data: Cleanup" {
        # "Cleanup any data and references, here.\n(this is called automatically, by the Macro: Exit)"
        n133 = Unbundle By Name(w342) -> ("Core.Current VI Reference"=w345:refnum<vi>)
        n134 = Close Reference(reference=w345, error in (no error)=w344) -> (error out=w343:errorcluster)
        n135 = call <vilib>:"Add State(s) to Queue__JKI_lib_State_Machine.vi"("State(s) in (\"\")"=w347) -> ("States Out"=w346:string)  [unwired: 14 in]
      }
      frame "---------- UI ----------" {
        # "Do not put any code in this frame.\n(It is a separator no-op. You can make a copy of this frame to create a new UI frame)"
        n136 = call <vilib>:"Add State(s) to Queue__JKI_lib_State_Machine.vi"("State(s) in (\"\")"=w354) -> ("States Out"=w353:string)  [unwired: 14 in]
      }
      frame "UI: Initialize" {
        # "Initialize the User Interface, here.\n(this is called automatically, by the Macro: Init)"
        n137 = Unbundle By Name(w358) -> ("Toolbar.Advance"=w357:refnum<vi>[])
        n138 = disable-structure shown="Disabled" {
          disable-tunnel: w357 -> [w364 _]
          frame Disabled {
            n139 = for {
              tunnel: w364 -> [w366] mode=indexing
              n140 = property class="Bool"(reference=w366, "Visible"=FALSE) -> ()  [unwired: 1 in, 2 out]
            }
          }
          frame Enabled {
          }
        }
        n141 = local write "Peroid Logs"(TRUE ("Filter Peroid Logs")) -> ()
        n142 = call <vilib>:"Add State(s) to Queue__JKI_lib_State_Machine.vi"("State(s) in (\"\")"=w363) -> ("States Out"=w362:string)  [unwired: 14 in]
      }
      frame "UI: Cursor Set" {
        # "Argument"
        # "Set and Unset Cursor Busy.\n(Usage: \"UI: Cursor Set >> Busy|Idle\")"
        n143 = case shown="\"Idle\", Default" w370 {
          tunnel: w372 -> [w377 w379]
          tunnel: [w376 w378] -> w371
          frame "Idle", Default {
            n144 = call <vilib>:"Unset Busy.vi"("error in (no error)"=w377) -> ("error out"=w376:errorcluster)  [unwired: 10 in]
          }
          frame "Busy" {
            n145 = call <vilib>:"Set Busy.vi"("error in (no error)"=w379) -> ("error out"=w378:errorcluster)  [unwired: 9 in, 1 out]
          }
        }
        n146 = call <vilib>:"Add State(s) to Queue__JKI_lib_State_Machine.vi"("State(s) in (\"\")"=w375) -> ("States Out"=w374:string)  [unwired: 14 in]
      }
      frame "UI: Front Panel State" {
        # "Argument"
        # "Set Front Panel Open or Closed\n(Usage: \"UI: Front Panel State >> Open|Close\")"
        n147 = Unbundle By Name(w385) -> ("Core.Current VI Reference"=w384:refnum<vi>)
        n148 = case shown="\"Minimize\", \"Minimized\"" w383 {
          tunnel: w387 -> [w395 w410 w421 w434 w447]
          tunnel: [w397 w411 w423 w436 w449] -> w386
          tunnel: w384 -> [w396 w408 w422 w435 w448]
          frame "Open", "Standard", Default {
            w390 = T6."Standard" ("State")
            n149 = property class="VI"(reference=w396, error in=w395) -> (reference out=w393:refnum<vi>, error out=w394:errorcluster, "FP.State"=w392:T6)
            n150 = Not Equal?(x=w392, y=w390) -> (x != y?=w391:bool)
            n151 = case shown="True" w391 {
              tunnel: [w401 w403] -> w397
              tunnel: w394 -> [w400 w403]
              tunnel: w393 -> [w399 _]
              tunnel: w390 -> [w398 _]
              frame True {
                n152 = invoke class="VI" method="FP.Open"(reference=w399, error in=w400, "Activate"=TRUE, "State"=w398) -> (error out=w401:errorcluster)  [unwired: 1 in, 4 out]
              }
              frame False {
              }
            }
          }
          frame "Close", "Closed" {
            n153 = property class="VI"(reference=w408, error in=w410) -> (reference out=w407:refnum<vi>, error out=w409:errorcluster, "FP.State"=w405:T6)
            n154 = Not Equal?(x=w405, y=T6."Closed" ("Front Panel Window:State")) -> (x != y?=w404:bool)
            n155 = case shown="True" w404 {
              tunnel: [w412 w415] -> w411
              tunnel: w409 -> [w412 w414]
              tunnel: w407 -> [_ w413]
              frame False {
              }
              frame True {
                n156 = invoke class="VI" method="FP.Close"(reference=w413, error in=w414) -> (error out=w415:errorcluster)  [unwired: 1 in, 2 out]
              }
            }
          }
          frame "Hidden", "Hide" {
            w416 = T6."Hidden" ("State")
            n157 = property class="VI"(reference=w422, error in=w421) -> (reference out=w419:refnum<vi>, error out=w420:errorcluster, "FP.State"=w418:T6)
            n158 = Not Equal?(x=w418, y=w416) -> (x != y?=w417:bool)
            n159 = case shown="True" w417 {
              tunnel: [w427 w428] -> w423
              tunnel: w420 -> [w426 w428]
              tunnel: w419 -> [w425 _]
              tunnel: w416 -> [w424 _]
              frame True {
                n160 = invoke class="VI" method="FP.Open"(reference=w425, error in=w426, "State"=w424) -> (error out=w427:errorcluster)  [unwired: 2 in, 4 out]
              }
              frame False {
              }
            }
          }
          frame "Minimize", "Minimized" {
            w429 = T6."Minimized" ("State")
            n161 = property class="VI"(reference=w435, error in=w434) -> (reference out=w432:refnum<vi>, error out=w433:errorcluster, "FP.State"=w431:T6)
            n162 = Not Equal?(x=w431, y=w429) -> (x != y?=w430:bool)
            n163 = case shown="True" w430 {
              tunnel: [w440 w441] -> w436
              tunnel: w433 -> [w439 w441]
              tunnel: w432 -> [w438 _]
              tunnel: w429 -> [w437 _]
              frame True {
                n164 = invoke class="VI" method="FP.Open"(reference=w438, error in=w439, "State"=w437) -> (error out=w440:errorcluster)  [unwired: 2 in, 4 out]
              }
              frame False {
              }
            }
          }
          frame "Maximize", "Maximized" {
            w442 = T6."Maximized" ("State")
            n165 = property class="VI"(reference=w448, error in=w447) -> (reference out=w445:refnum<vi>, error out=w446:errorcluster, "FP.State"=w444:T6)
            n166 = Not Equal?(x=w444, y=w442) -> (x != y?=w443:bool)
            n167 = case shown="True" w443 {
              tunnel: [w453 w454] -> w449
              tunnel: w446 -> [w452 w454]
              tunnel: w445 -> [w451 _]
              tunnel: w442 -> [w450 _]
              frame True {
                n168 = invoke class="VI" method="FP.Open"(reference=w451, error in=w452, "State"=w450) -> (error out=w453:errorcluster)  [unwired: 2 in, 4 out]
              }
              frame False {
              }
            }
          }
        }
        n169 = call <vilib>:"Add State(s) to Queue__JKI_lib_State_Machine.vi"("State(s) in (\"\")"=w389) -> ("States Out"=w388:string)  [unwired: 14 in]
      }
      frame "UI: Update Broadcast Registry" {
        n170 = call "CSM - List Mapping Relationships in Broadcast Registry.vi"() -> ("Mapping Relationships"=w456:T13)  [unwired: 10 in, 1 out]
        n171 = for {
          tunnel: w456 -> [w470] mode=indexing
          tunnel: [w463] -> w457 mode=indexing
          n172 = Unbundle(w470) -> (w469:string, "Name"=w468:string, "Target CSM"=w467:string, "Target State"=w466:string, "Register Type"=w465:T12)
          n173 = Format Into String(w465) -> (resulting string=w464:string)  [unwired: 3 in, 1 out]
          n174 = Build Array(w469, w468, w467, w466, w464) -> (w463:string[])
        }
        "Broadcast Registry" <- w457
      }
      frame "UI: Update Toolbar" {
        w479 = i16 2 ("x")
        n175 = control-ref of="Record.Start"() -> (w487:refnum<vi>)
        n176 = control-ref of="Record.Stop"() -> (w486:refnum<vi>)
        n177 = Unbundle By Name(w485) -> ("Core.Current VI Reference"=w476:refnum<vi>, "LogFile"=w473:path, "LoggerWatchDogQueue"=w484:refnum<queue>)
        n178 = Not A Number/Path/Refnum?(number/path/refnum=w484) -> (NaN/Path/Refnum?=w477:bool)
        n179 = Not(x=w477) -> (.not. x?=w478:bool)
        n180 = Boolean To (0,1)(Boolean=w478) -> (0, 1=w483:i16)
        n181 = Boolean To (0,1)(Boolean=w477) -> (0, 1=w482:i16)
        n182 = Multiply(x=w479, y=w482) -> (x*y=w480:i16)
        n183 = Multiply(x=w479, y=w483) -> (x*y=w481:i16)
        n184 = Empty String/Path?(string/path=w473) -> (empty?=w472:bool)
        n185 = property class="Bool"(reference=w487, "DisabledEnum"=w481) -> ()  [unwired: 1 in, 2 out]
        n186 = property class="Bool"(reference=w486, "DisabledEnum"=w480) -> ()  [unwired: 1 in, 2 out]
        n187 = case shown="True" w472 {
          tunnel: "Running Log Viewer (CSM)" ("Front Panel Window:Title") -> [w496 w497]
          tunnel: [w495 w497] -> w474
          tunnel: w473 -> [w492 _]
          frame False {
            n188 = Path To String(path=w492) -> (string=w493:string)
            n189 = Concatenate Strings(w496, " - " ("string"), w493) -> (w495:string)
          }
          frame True {
          }
        }
        n190 = property class="VI"(reference=w476, "Front Panel.Title"=w474) -> ()  [unwired: 1 in, 2 out]
      }
      frame "UI: Resize Tab Content" {
        n191 = control-ref of="Tab"() -> (w502:refnum<vi>)
        n192 = invoke class="TabCtl (strict)" method="FitControlToPane"(reference=w502) -> (reference out=w501:refnum<vi>)  [unwired: 2 in, 2 out]
        n193 = control-ref of="Broadcast Registry"() -> (w500:refnum<vi>)
        n194 = control-ref of="Error History"() -> (w499:refnum<vi>)
        n195 = Build Array(w500, w499) -> (w498:refnum<vi>[])
        n196 = for {
          tunnel: w501 -> [w510]
          tunnel: w498 -> [w509] mode=indexing
          n197 = call "Fit Control to Tab.vi"("Control"=w509, "TabRef"=w510) -> ()  [unwired: 5 in, 3 out]
        }
      }
      frame "---------- Macro ----------" {
        # "Do not put any code in this frame.\n(It is a separator no-op. You can make a copy of this frame to create a new Macro frame)"
        n198 = call <vilib>:"Add State(s) to Queue__JKI_lib_State_Machine.vi"("State(s) in (\"\")"=w517) -> ("States Out"=w516:string)  [unwired: 14 in]
      }
      frame "Macro: Initialize" {
        w521 = "Data: Initialize\nData: Initialize References\nInitialize Core Data\nUI: Initialize\nUI: Front Panel State >> Open\nUI: Resize Tab Content\nUI: Update Broadcast Registry\nUI: Update Toolbar"  # Data: Initialize Data: Initialize References Initialize Core Data UI: Initialize UI: Front Panel State >> Open UI: Resize Tab Content UI: Update Broadcast Registry UI: Update Toolbar
        # "Initialization Macro\n(This is called once, when the VI starts)"
        n199 = call <vilib>:"Add State(s) to Queue__JKI_lib_State_Machine.vi"("State(s) in Front (\"\")"=w521, "State(s) in (\"\")"=w525) -> ("States Out"=w524:string)  [unwired: 13 in]
      }
      frame "Macro: Exit" {
        # "Exit Macro\n(This is called once, when the VI exits)"
        n200 = call <vilib>:"Add State(s) to Queue__JKI_lib_State_Machine.vi"("State(s) at Back (\"\")"="Data: Cleanup\nExit") -> ("States Out"=w529:string)  [unwired: 14 in]
        n201 = call <vilib>:"Add State(s) to Queue__JKI_lib_State_Machine.vi"("State(s) in Front (\"\")"=w529, "State(s) in (\"\")"=w534) -> ("States Out"=w533:string)  [unwired: 13 in]
      }
    }
  }
  n202 = disable-structure shown="Disabled" {
    frame Disabled {
      n203 = call "CSM - Module VI Reference.vi"("Response Timeout (-2 Using Global Settings)"=1000 ("Response Timeout(5000 ms)"), "error in (no error)"=errorcluster {"status"=FALSE, "code"=0, "source"=""}, "CSM Name"="") -> ("error out"=w541:errorcluster, "CSM Module VIRef"=w540:refnum<vi>)  [unwired: 7 in]
      n204 = invoke on="Invoke Node" class="VI" method="FP.Open"(reference=w540, error in=w541, "Activate"=TRUE ("Activate?")) -> (error out=w539:errorcluster)  [unwired: 2 in, 4 out]
      n205 = call <vilib>:"Simple Error Handler.vi"("error in (no error)"=w539) -> ()  [unwired: 4 in, 5 out]
    }
    frame Enabled {
    }
  }
  n206 = flat-sequence {
    tunnel: [w543] -> w8
    tunnel: w7 -> [w543]
    frame #0 {
      n207 = local write "Stop"(TRUE ("Stop")) -> ()
    }
  }
  n208 = call "CSM - Destroy Global Log Queue.vi"("Error In"=w25, "Global Log Queue"=w23) -> ("error out"=w9:errorcluster)  [unwired: 9 in]
  n209 = Merge Errors(w8, w9) -> (w10:errorcluster)
  n210 = Destroy User Event(user event=w11, error in=w10) -> (error out=w5:errorcluster)
  n211 = control-ref of="Current VI Reference"() -> (w3:refnum<vi>)
  n212 = call "Close FP if in LabVIEW Dir.vi"("VI Refnum"=w3, "Error in"=w5) -> ("Error out"=w4:errorcluster)  [unwired: 9 in]
  n213 = call <vilib>:"Clear Errors.vi"("error in (no error)"=w4) -> ()  [unwired: 5 in, 2 out]
